vi "request SCPI Command.vi"(8 "error in (no error)":errorcluster, 10 "SCPI Command":string, 11 "NR in":refnum<class "NR.lvclass">) -> (0 "error out":errorcluster, 3 "NR out":refnum<class "NR.lvclass">)   [LabVIEW 2023, in "ANRITSU Call Box.lvlib" / "NR.lvclass"]
uses:
  NR.lvclass
  NR.lvclass/NR.ctl
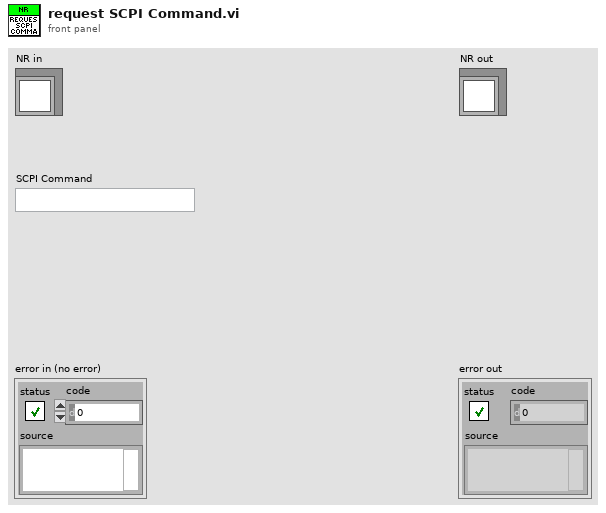
[diagram p1: front panel]
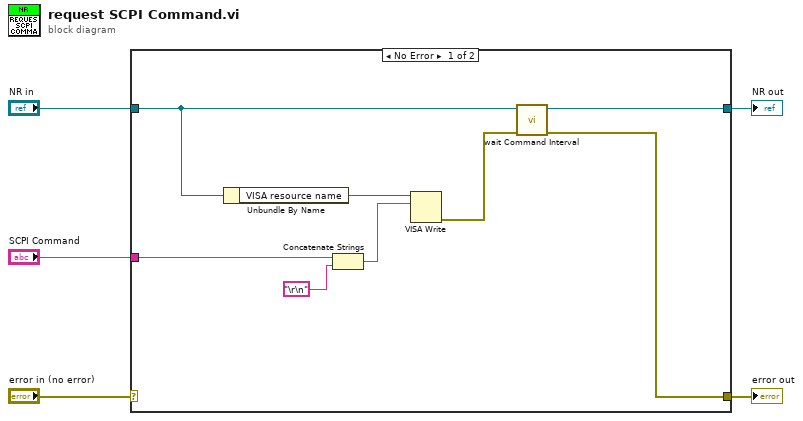
[diagram p0: block diagram]
diagram:
  n1 = case shown="No Error" "error in (no error)" {
    selector: "error in (no error)" -> [_ w15]
    tunnel: [w6 w15] -> w4
    tunnel: [w8 w14] -> w2
    tunnel: "NR in" -> [w9 w14]
    tunnel: "SCPI Command" -> [w12 _]
    frame No Error {
      n2 = Unbundle By Name(w9) -> ("VISA resource name"=w13:refnum<visa-resource-name>)
      n3 = Concatenate Strings(w12, "\r\n") -> (w10:string)
      n4 = VISA Write(VISA resource name=w13, write buffer=w10) -> (error out=w7:errorcluster)  [unwired: 1 in, 2 out]
      n5 = call "wait Command Interval.vi"("error in (no error)"=w7, "NR in"=w9) -> ("error out"=w6:errorcluster, "NR out"=w8:refnum<class "NR.lvclass">)  [unwired: 8 in]
    }
    frame Error {
    }
  }
  "error out" <- w4
  "NR out" <- w2
